vi "Test - Check All.vi"(8 "error in":errorcluster, 9 "Conditions":bool[](array[boolean]), 10 "Check Names":string[](array[string]), 11 "Report in":string) -> (0 "error out":errorcluster, 3 "Report out":string)   [LabVIEW 2026]
doc: "Test helper. Runs Test - Check.vi once per element of Conditions, with the Check Name at the same index, and appends one PASS or FAIL line per check to Report. Lets a test VI collect all its conditions with Build Array and report them in one call. A missing name is reported as an empty name. error in is passed through unchanged.\n\nGenerated by: Claude"
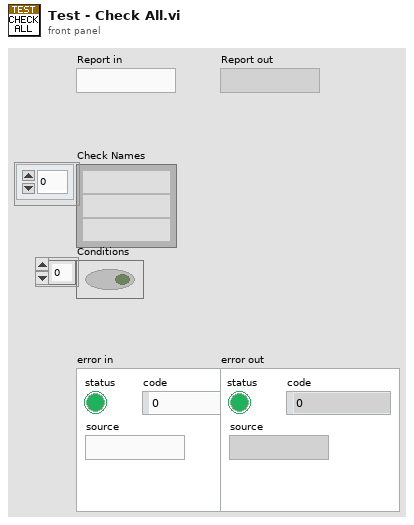
[diagram p1: front panel]
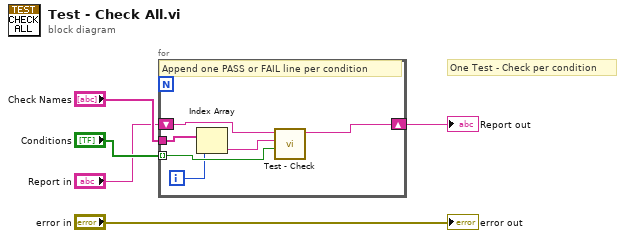
[diagram p0: block diagram]
diagram:
  # "One Test - Check per condition"
  n1 = for {
    tunnel: "Conditions" -> [w7] mode=indexing
    tunnel: "Check Names" -> [w8]
    shift-right: [w10] -> w5
    shift-left: "Report in" -> [w9]
    i -> [w6]
    # "Append one PASS or FAIL line per condition"
    n2 = Index Array(array=w8, index=w6) -> (element=w11:string)
    n3 = call "Test - Check.vi"("Condition"=w7, "Check Name"=w11, "Report in"=w9) -> ("Report out"=w10:string)  [unwired: 7 in, 1 out]
  }
  "Report out" <- w5
  "error out" <- "error in"
